vi "Untitled 2.vi"(4 "User Parameter":variant, 5 "Event Data":cluster{"e":refnum<k24>}, 6 "Control Ref":refnum<k24>, 7 "Event Common Data":T1) -> ()   [LabVIEW 2026]
uses:
  C:/Users/loicw/Documents/LabVIEW/ToastNotifications/Sources/bins/Microsoft.Toolkit.Uwp.Notifications.dll
  bins/Microsoft.Toolkit.Uwp.Notifications.dll
  C:/Users/loicw/Documents/LabVIEW/ToastNotifications/Sources/SandBox/Untitled 2.vi/Windows.Foundation
  Windows.Foundation
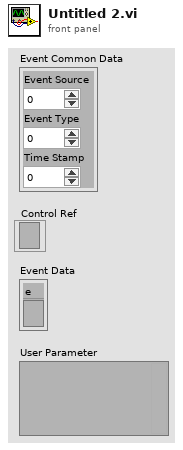
[diagram p1: front panel]
types:
  T1 = cluster{"Event Source":i32, "Event Type":u32, "Time Stamp":u32}
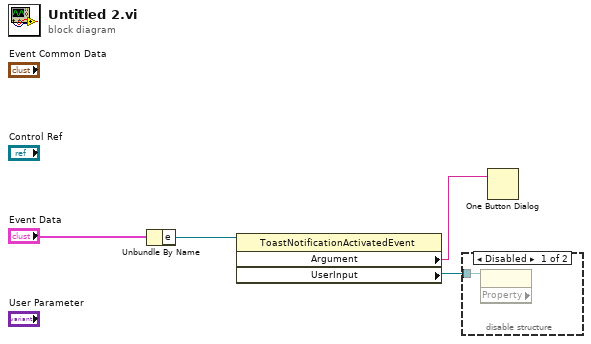
[diagram p0: block diagram]
diagram:
  n1 = Unbundle By Name("Event Data") -> ("e"=w3:refnum<k24>)
  n2 = property class="ToastNotificationActivatedEvent"(reference=w3) -> ("Argument"=w1:string, "UserInput"=w2:refnum<k24>)  [unwired: 1 in, 2 out]
  n3 = disable-structure shown="Disabled" {
    disable-tunnel: w2 -> [w5 _]
    frame Disabled {
      n4 = property props=[](reference=w5) -> ()  [unwired: 1 in, 3 out]
    }
    frame Enabled {
    }
  }
  n5 = One Button Dialog(message=w1) -> ()  [unwired: 1 in, 1 out]
